vi "VisionTrig.vi"(8 "(F) 4Final distance away from the target to end":dbl format="%#_13g", 9 "(Omega) difference in heading between robot and target's perpindicular line":dbl format="%#_13g", 10 "(I) Vision's distance to target":dbl format="%#_13g", 11 "(phi) Vision's angle that the target is offcenter":dbl format="%#_13g") -> (1 "3Angle to turn to be perpindicular to the target":dbl, 2 "2Distance to drive":dbl, 3 "1 Angle to turn to get to the destination point":dbl)   [LabVIEW 2018]
panel:
  out "Epsilon":dbl
  out "Theta":dbl
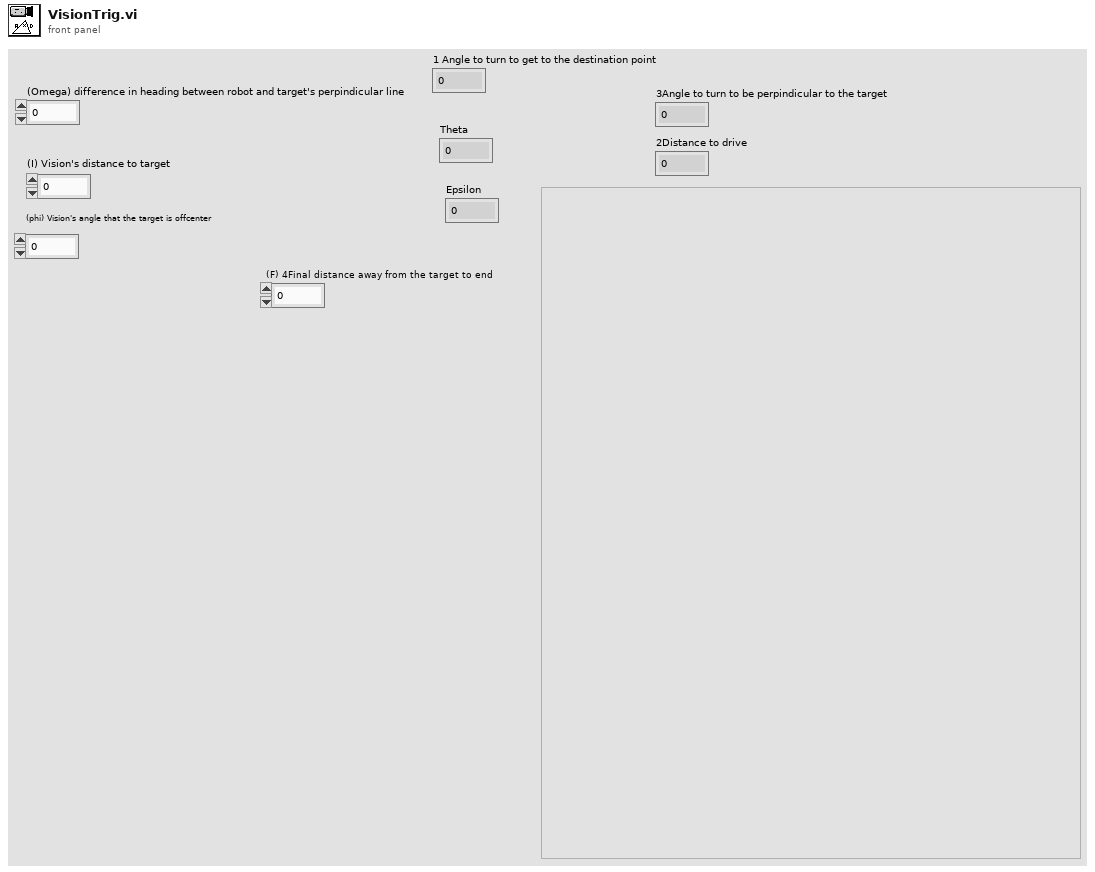
[diagram p1: front panel]
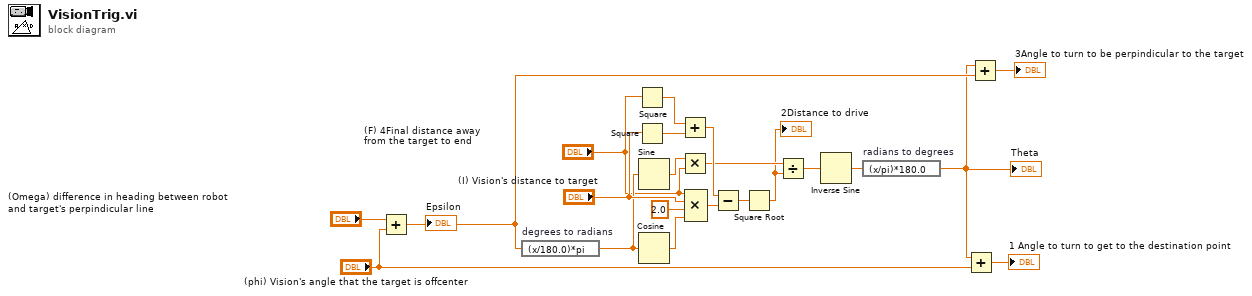
[diagram p0: block diagram]
diagram:
  n1 = Add(x="(Omega) difference in heading between robot and target's perpindicular line", y="(phi) Vision's angle that the target is offcenter") -> (x+y=w5:dbl)
  "Epsilon" <- w5
  n2 = expression code="(x/180.0)*pi" "degrees to radians"(w5) -> (w12:dbl)
  n3 = Square(x="(F) 4Final distance away from the target to end") -> (x^2=w20:dbl)
  n4 = Square(x="(I) Vision's distance to target") -> (x^2=w19:dbl)
  n5 = Sine(x=w12) -> (sin(x)=w11:dbl)
  n6 = Cosine(x=w12) -> (cos(x)=w15:dbl)
  n7 = Add(x=w20, y=w19) -> (x+y=w18:dbl)
  n8 = Multiply(x=w11, y="(F) 4Final distance away from the target to end") -> (x*y=w9:dbl)
  n9 = Compound Arithmetic op=MULTIPLY("(F) 4Final distance away from the target to end", "(I) Vision's distance to target", 2.0 ("value"), w15) -> (w14:dbl)
  n10 = Subtract(x=w18, y=w14) -> (x-y=w13:dbl)
  n11 = Square Root(x=w13) -> (sqrt(x)=w8:dbl)
  "2Distance to drive" <- w8
  n12 = Divide(x=w9, y=w8) -> (x/y=w7:dbl)
  n13 = Inverse Sine(1:w7) -> (0:w6:dbl)
  n14 = expression code="(x/pi)*180.0" "radians to degrees"(w6) -> (w3:dbl)
  "Theta" <- w3
  n15 = Add(x=w3, y="(phi) Vision's angle that the target is offcenter") -> (x+y=→"1 Angle to turn to get to the destination point":dbl)
  n16 = Add(x=w3, y=w5) -> (x+y=→"3Angle to turn to be perpindicular to the target":dbl)
